vi "Tell Parent.vi"(4 "Priority":bool, 7 "Actor in":refnum<class "Actor.lvclass">, 8 "Error in":errorcluster, 9 "Reply":bool, 10 "Msg":refnum<class "Msg.lvclass">) -> (0 "Error out":errorcluster, 5 "Actor out":refnum<class "Actor.lvclass">)   [LabVIEW 2020, in "jettl.lvlib"]
uses:
  jettl.lvlib
  Msg/Msg.lvclass
  Actor/Actor.lvclass
  Relation.ctl
  Base Teller/Base Teller/Base Teller.lvclass/Base Teller.ctl
  Base Teller/Init Teller.vi
  Default Implementation.vi
  Base Teller/Base Teller/Init Teller.vi
  Base Teller/Base Teller/Base Teller.lvclass
  C:/git/jettl/src/jettl/jettl/Teller/Teller.lvclass
  Attributes/Attributes.lvclass
  Msg Input/Msg Input.lvclass
  Transport/Transport.lvclass
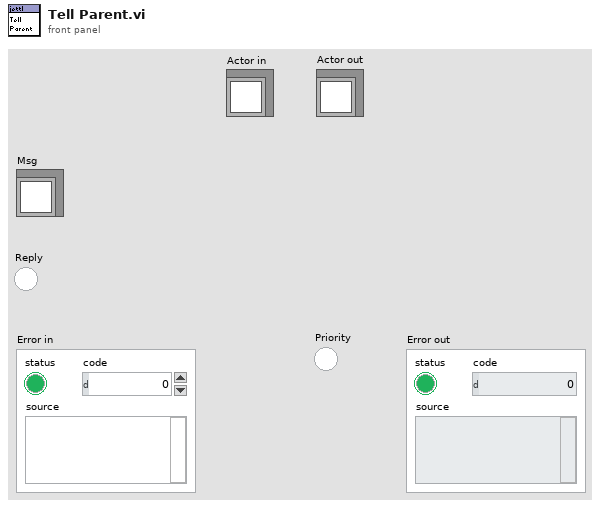
[diagram p1: front panel]
types:
  T1 = typedef "jettl.lvlib/Relation.ctl" = enum16{"Self", "Parent", "Child", "No Relation"}
  T2 = typedef "jettl.lvlib/Msgs.ctl" = set{refnum<class "Msg.lvclass">}
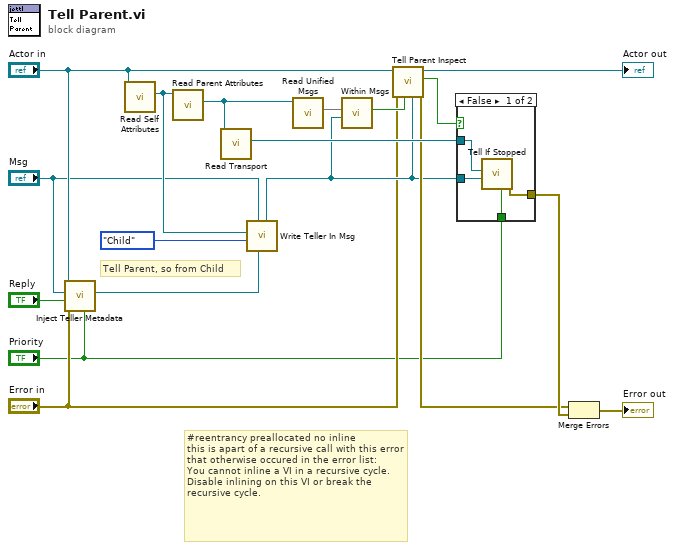
[diagram p0: block diagram]
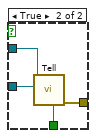
[diagram p2: hidden frame]
diagram:
  # "#reentrancy preallocated no inline\nthis is apart of a recursive call with this error that otherwise occured in the error list:\nYou cannot inline a VI in a recursive cycle. Disable inlining on this VI or break the recursive cycle."
  # "Tell Parent, so from Child"
  n1 = call-dynamic "Inject Teller Metadata.vi"("Priority"="Priority", "Error in"="Error in", "Reply"="Reply", "Msg"="Msg", "Actor in"="Actor in") -> ("Teller Metadata"=w5:refnum<class "Teller Metadata.lvclass">)  [unwired: 6 in]
  n2 = call-dynamic "Read Self Attributes.vi"("Actor in"="Actor in") -> ("Self Attributes"=w12:refnum<class "Attributes.lvclass">)  [unwired: 10 in]
  n3 = call-dynamic "Read Parent Attributes.vi"("Attributes in"=w12) -> ("Parent Attributes"=w10:refnum<class "Attributes.lvclass">)  [unwired: 10 in]
  n4 = call-dynamic "Read Transport.vi"("Attributes in"=w10) -> ("Transport"=w17:refnum<class "Transport.lvclass">)  [unwired: 10 in]
  n5 = call "Write Teller In Msg.vi"("Teller Metadata"=w5, "Msg in"="Msg", "Relation"=Relation."Child", "Attributes"=w12) -> ("Msg out"=w8:refnum<class "Msg.lvclass">)  [unwired: 7 in]
  n6 = call-dynamic "Read Unified Msgs.vi"("Attributes in"=w10) -> ("Unified Msgs"=w11:T2)  [unwired: 10 in]
  n7 = call "Within Msgs.vi"("Msg"=w8, "Msgs"=w11) -> ("Within Msgs"=w9:bool)  [unwired: 9 in]
  n8 = call-dynamic "Tell Parent Inspect.vi"("Msg"=w8, "Within Unified Msgs"=w9, "Error in"="Error in", "Actor in"="Actor in") -> ("Error out"=w13:errorcluster, "Proceed"=w7:bool, "Actor out"=→"Actor out":refnum<class "Actor.lvclass">)  [unwired: 5 in]
  n9 = case shown="False" w7 {
    tunnel: [w20 w26] -> w18
    tunnel: w17 -> [w19 w25]
    tunnel: "Priority" -> [w21 w24]
    tunnel: w8 -> [w22 w23]
    frame False {
      n10 = call "Tell If Stopped.vi"("Priority"=w21, "Msg"=w22, "Transport"=w19) -> ("Error out"=w20:errorcluster)  [unwired: 8 in]
    }
    frame True {
      n11 = call-dynamic "Tell.vi"("Priority"=w24, "Msg"=w23, "Transport in"=w25) -> ("Error out"=w26:errorcluster)  [unwired: 8 in]
    }
  }
  n12 = Merge Errors(w13, w18) -> (→"Error out":errorcluster)
